vi "Measurement Logic.vi"() -> ()   [LabVIEW 2022 SP3, in "Noise Sweep_Class D Amplifier.lvlib"]
uses:
  Noise Sweep_Class D Amplifier.lvlib
  <vilib>/Analysis/NI_AALBase.lvlib
  <instrlib>/niDCPower/nidcpower.llb/niDCPower Source Mode.ctl
  <instrlib>/niDCPower/nidcpower.llb/niDCPower Output Function.ctl
  Measurement Results.ctl
  <instrlib>/niDCPower/nidcpower.llb/niDCPower Wait For Event - Event.ctl
  <vilib>/Analysis/NI_AALPro.lvlib
  shared/DAQmx/DAQmx utility.lvlib
  shared/digital serial api/Digital Serial.lvclass
  shared/digital serial gen settings/digital audio protocol controls.lvlib
  shared/controls/digital output level units.ctl
  shared/controls/audio controls.lvlib
  service/generation/controls/sine wave properties.ctl
  service/generation/controls/AudioGenTypeDefs.lvlib
  shared/controls/weighting filter.ctl
  shared/controls/highpass filter.ctl
  shared/controls/lowpass filter.ctl
  shared/controls/audio filter settings.ctl
  <vilib>/DAQmx/configure/timing.llb/DAQmx Timing (Sample Clock).vi
  <vilib>/DAQmx/create/channels.llb/DAQmx Create Channel (AI-Voltage-Basic).vi
  <vilib>/Analysis/1siggen.llb/Ramp Pattern by Samples.vi
  <vilib>/Analysis/5stat.llb/RMS (DBL).vi
  <vilib>/Plug-In SDKs/Measurements/Measure Call Context/Measure Call Context.lvclass
  Measurement Configuration.ctl
  shared/DAQmx/input terminal configuration.ctl
panel:
  out "XY Graph":cluster{"X data":dbl[], "Y data":dbl[]}[](graph)
  out "Waveform Graph":waveform(dbl)[](graph)
  out "measure call context out":refnum<class "Measure Call Context.lvclass">
  in  "measure call context in":refnum<class "Measure Call Context.lvclass">
  out "measurement results":T1={"channel names"=[], "power supply voltage (V)"=[], "idle channel noise (Vrms)"=[], "wfm - dt"=1.9531249997269942e-05, "wfm - data"=array[12800 elements]}
  in  "measurement configuration":T2={"digital serial cfg file"="", "digital channel list"="7821\\PCMo 8", "master clock channel list"="7821\\PCMo 0", "acq channel"="PXI1Slot4/ai0", "acq sampling rate"=51200.0, "measurement time (s)"=0.1, "delay before measurement (s)"=0.1, "input range"=5.0, "input terminal cfg"=enum."Default", "weighting filter"=enum."A-weighting", "lowpass filter"=enum."No filter", "highpass filter"=enum."DC", "power supply resource"="PXI1Slot6", "power supply voltage start"=5.0, "power supply voltage stop"=14.0, "sweep number of steps"=10, "power supply current limit"=1.2}
  out "error out":errorcluster
  in  "error in":errorcluster
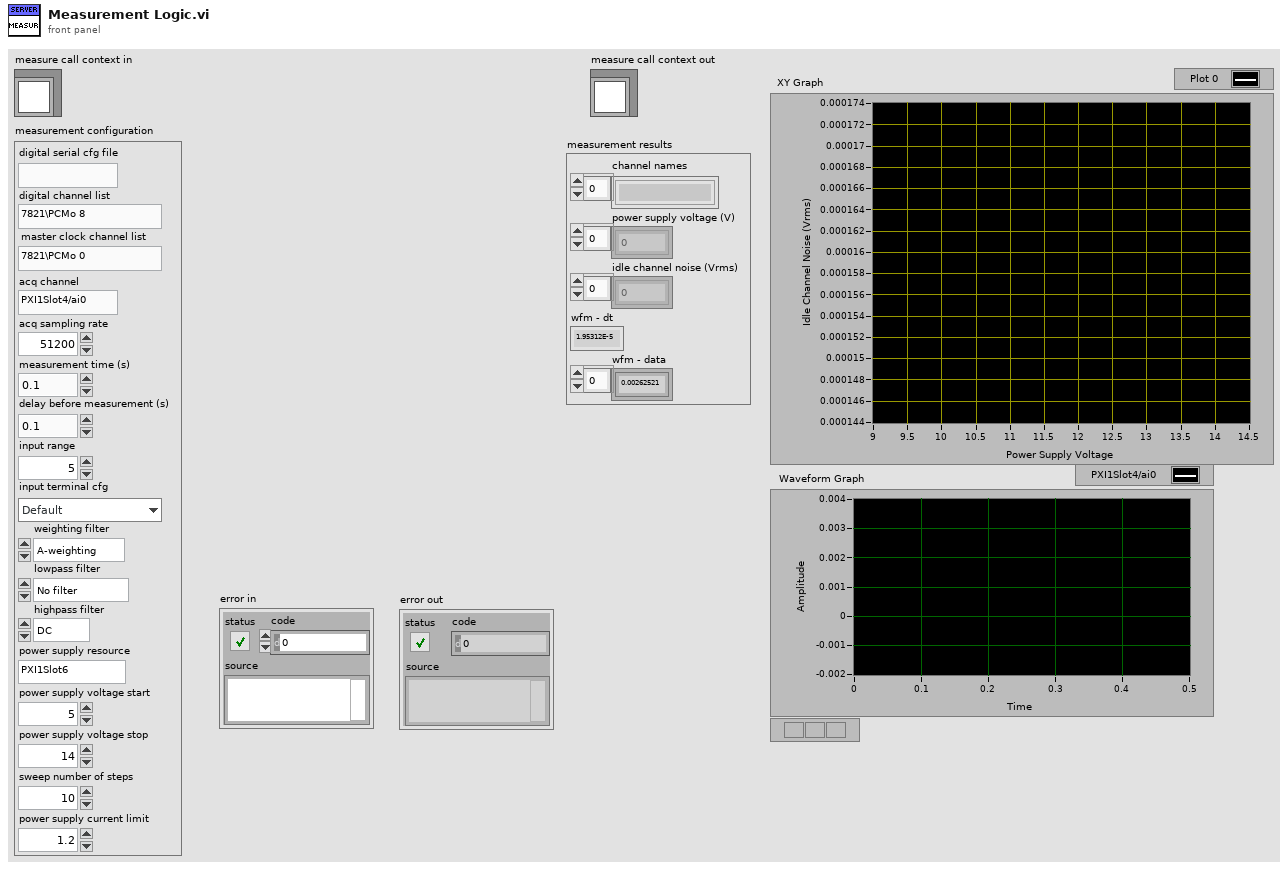
[diagram p1: front panel]
types:
  T1 = typedef "Noise Sweep_Class D Amplifier.lvlib/Measurement Results.ctl" = cluster{"channel names":string[], "power supply voltage (V)":dbl[], "idle channel noise (Vrms)":dbl[], "wfm - dt":dbl, "wfm - data":dbl[]}
  T2 = typedef "Noise Sweep_Class D Amplifier.lvlib/Measurement Configuration.ctl" = cluster{"digital serial cfg file":string, "digital channel list":string, "master clock channel list":string, "acq channel":string, "acq sampling rate":dbl, "measurement time (s)":dbl, "delay before measurement (s)":dbl, "input range":dbl, "input terminal cfg":T3, "weighting filter":T4, "lowpass filter":T5, "highpass filter":T6, "power supply resource":string, "power supply voltage start":dbl, "power supply voltage stop":dbl, "sweep number of steps":u32, "power supply current limit":dbl}
  T3 = typedef "DAQmx utility.lvlib/input terminal configuration.ctl" = enum32{"Default", "NRSE", "RSE", "Differential", "Pseudodifferential"}
  T4 = typedef "weighting filter.ctl" = enum32{"Linear", "A-weighting", "B-weighting", "C-weighting"}
  T5 = typedef "lowpass filter.ctl" = enum32{"No filter", "AES17 20kHz", "AES17 40kHz"}
  T6 = typedef "highpass filter.ctl" = enum32{"DC", "AC"}
  T7 = typedef "audio filter settings.ctl" = cluster{"weighting filter":T4, "highpass filter":T6, "lowpass filter ":T5}
  T8 = typedef "AudioGenTypeDefs.lvlib/sine wave properties.ctl" = cluster{"frequency":dbl, "amplitude":dbl, "phase":dbl}[]
  T9 = typedef "audio controls.lvlib/digital output level units.ctl" = enum32{"% FS", "dBFS", "V"}
  T10 = typedef "niDCPower Output Function.ctl" = i32
  T11 = typedef "niDCPower Source Mode.ctl" = i32
  T12 = typedef "digital serial gen settings.ctl" = cluster{"number of channels":u32, "data justification":T13, "endianness":T14, "channel length":u32, "bit depth":u32, "frame clock rate":dbl, "bit clock edge sync":T15, "master clock rate":dbl, "Logic Level":T16, "frame sync edge for channel 0":T15, "Channel 0 Offset":u32}
  T13 = typedef "PDM Shared.lvlib/PCM Data Justification.ctl" = enum16{"Left Justified", "Right Justified"}
  T14 = typedef "PDM Shared.lvlib/PCM Bit Endianness.ctl" = enum16{"MSB First", "LSB First"}
  T15 = typedef "PDM Shared.lvlib/Digital Edge.ctl" = enum8{"Rising", "Falling"}
  T16 = typedef "PDM Acquisition Class Library.lvlib/DecoderSession.lvclass/Logic Levels.ctl" = enum16{"3.3 V", "1.8 V", "1.2 V"}
  T17 = typedef "AudioGenTypeDefs.lvlib/digital protocol settings.ctl" = cluster{"logic level":T16, "PCM Data Configuration":T18, "bit clock rate":sgl, "master clock rate":sgl, "clock mode":T19, "Frame Sync Clock Control":T20}
  T18 = typedef "PDM Shared.lvlib/PCM Data Format Configuration.ctl" = cluster{"Frame Sync Edge for Channel 0":T15, "Channel Count Per Frame":u8, "Channel Length":u16, "Bit Depth":u8, "Channel 0 Offset":u16, "Endianness":T14, "Data Justification":T13}
  T19 = typedef "PDM Shared.lvlib/clock mode.ctl" = enum16{"divided clock", "DDS"}
  T20 = typedef "PDM Shared.lvlib/PCM Frame Sync Control.ctl" = cluster{"Frame Length":u16, "Frame Sync Pulse Width":u16, "Bit Clock Edge  Sync":T15}
  T21 = typedef "niDCPower Wait For Event - Event.ctl" = i32
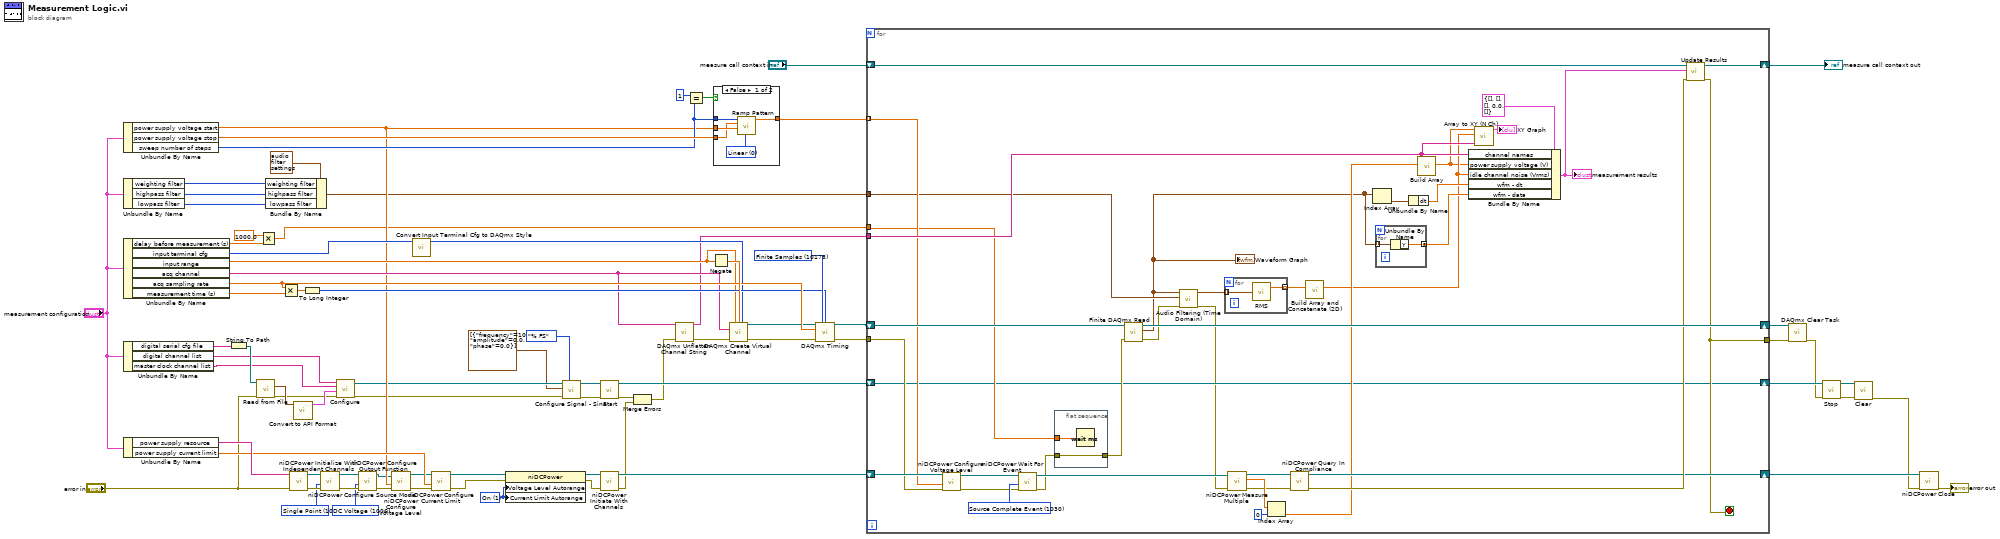
[diagram p0: block diagram]
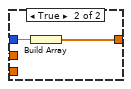
[diagram p2: hidden frame]
diagram:
  w33 = 1 items=["Off", "On"] ("Source:DC Voltage:Current Limit Autorange")
  w34 = T10 1006 items=["DC Voltage"=1006, "DC Current"=1007, "Pulse Voltage"=1049, "Pulse Current"=1050] ("output function")
  w41 = T11 1020 items=["Single Point"=1020, "Sequence"=1021] ("source mode")
  w65 = 10178 items=["Finite Samples"=10178, "Continuous Samples"=10123, "Hardware Timed Single Point"=12522] ("sample mode")
  n1 = Unbundle By Name("measurement configuration") -> ("power supply voltage start"=w49:dbl, "power supply voltage stop"=w68:dbl, "sweep number of steps"=w67:u32)
  n2 = Unbundle By Name("measurement configuration") -> ("weighting filter"=w4:T4, "highpass filter"=w3:T6, "lowpass filter"=w2:T5)
  n3 = Unbundle By Name("measurement configuration") -> ("delay before measurement (s)"=w32:dbl, "input terminal cfg"=w57:T3, "input range"=w59:dbl, "acq channel"=w51:string, "acq sampling rate"=w63:dbl, "measurement time (s)"=w64:dbl)
  n4 = Unbundle By Name("measurement configuration") -> ("digital serial cfg file"=w26:string, "digital channel list"=w19:string, "master clock channel list"=w18:string)
  n5 = Unbundle By Name("measurement configuration") -> ("power supply resource"=w73:string, "power supply current limit"=w72:dbl)
  n6 = String To Path(string=w26) -> (path=w25:path)
  n7 = call "Read from File.vi"("error in (no error)"="error in", "file path"=w25) -> ("error out"=w24:errorcluster, "digital audio protocol settings"=w29:T12)  [unwired: 7 in, 1 out]
  n8 = Multiply(x=1000.0, y=w32) -> (x*y=w30:dbl)
  n9 = Bundle By Name(cluster=T7 {"weighting filter"=enum."C-weighting", "highpass filter"=enum."AC", "lowpass filter "=enum."AES17 20kHz"} ("filter settings"), "weighting filter"=w4, "highpass filter"=w3, "lowpass filter"=w2) -> (w1:T7)
  n10 = Multiply(x=w63, y=w64) -> (x*y=w62:dbl)
  n11 = call <instrlib>:"niDCPower Initialize With Independent Channels.vi"("error in (no error)"="error in", "resource name"=w73) -> ("error out"=w45:errorcluster, "instrument handle out"=w44:refnum<k15>)  [unwired: 8 in]
  n12 = call "Convert to API Format.vi"("digital audio protocol settings"=w29) -> ("digital protocol settings"=w28:T17)  [unwired: 10 in]
  n13 = To Long Integer(number=w62) -> (32bit integer=w61:i32)
  n14 = call <instrlib>:"niDCPower Configure Source Mode.vi"("error in (no error)"=w45, "source mode"=w41, "instrument handle"=w44) -> ("error out"=w43:errorcluster, "instrument handle out"=w42:refnum<k15>)  [unwired: 7 out]
  n15 = call "Configure.vi"("error in (no error)"=w24, "digital protocol settings"=w28, "master clock channel list"=w18, "data channel list"=w19) -> ("error out"=w23:errorcluster, "digital serial task"=w22:refnum<class "Digital Serial.lvclass">)  [unwired: 6 in]
  n16 = call <instrlib>:"niDCPower Configure Output Function.vi"("error in (no error)"=w43, "output function"=w34, "instrument handle"=w42) -> ("error out"=w35:errorcluster, "instrument handle out"=w36:refnum<k15>)  [unwired: 1 in, 6 out]
  n17 = call <instrlib>:"niDCPower Configure Voltage Level.vi"("error in (no error)"=w35, "voltage level"=w49, "instrument handle"=w36) -> ("error out"=w46:errorcluster, "instrument handle out"=w47:refnum<k15>)  [unwired: 1 in, 6 out]
  n18 = call "Convert Input Terminal Cfg to DAQmx Style.vi"("input terminal cfg"=w57) -> ("DAQmx input terminal cfg"=w58:i32)  [unwired: 10 in]
  n19 = call <instrlib>:"niDCPower Configure Current Limit.vi"("error in (no error)"=w46, "current limit"=w72, "instrument handle"=w47) -> ("error out"=w37:errorcluster, "instrument handle out"=w40:refnum<k15>)  [unwired: 2 in, 5 out]
  n20 = property class="niDCPower"(reference=w40, error in=w37, "Voltage Level Autorange"=w33, "Current Limit Autorange"=w33) -> (reference out=w39:refnum<k15>, error out=w38:errorcluster)
  n21 = call "Configure Signal - Sine.vi"("output level units"=digital_output_level_units."% FS", "error in (no error)"=w23, "sine wave properties"=T8 [{"frequency"=1000.0, "amplitude"=0.0, "phase"=0.0}], "Digital Serial in"=w22) -> ("error out"=w20:errorcluster, "Digital Serial out"=w21:refnum<class "Digital Serial.lvclass">)  [unwired: 6 in]
  n22 = call <instrlib>:"niDCPower Initiate With Channels.vi"("error in (no error)"=w38, "instrument handle"=w39) -> ("error out"=w16:errorcluster, "instrument handle out"=w48:refnum<k15>)  [unwired: 8 in]
  n23 = call "Start.vi"("error in (no error)"=w20, "Digital Serial in"=w21) -> ("error out"=w15:errorcluster, "Digital Serial out"=w17:refnum<class "Digital Serial.lvclass">)  [unwired: 8 in]
  n24 = Merge Errors(w15, w16) -> (w14:errorcluster)
  n25 = call <vilib>:"DAQmx Unflatten Channel String.vi"("names in"=w51, "error in"=w14) -> ("names out"=w50:string[], "error out"=w52:errorcluster)  [unwired: 12 in]
  n26 = Equal?(x=u32 1, y=w67) -> (x = y?=w76:bool)
  n27 = Negate(x=w59) -> (-x=w66:dbl)
  n28 = case shown="False" w76 {
    tunnel: w49 -> [w83 w85]
    tunnel: w68 -> [w82 _]
    tunnel: w67 -> [w81 _]
    tunnel: [w80 w84] -> w78
    frame False {
      w79 = u16 0 items=["Linear", "Logarithmic"] ("type")
      n29 = call-poly <vilib>:"Ramp Pattern.vi"("type"=w79, "start"=w83, "end"=w82, "samples"=w81) -> ("Ramp Pattern"=w80:dbl[])  [unwired: 6 in, 1 out]
    }
    frame True {
      n30 = Build Array(w85) -> (w84:dbl[])
    }
  }
  n31 = call-poly <vilib>:"DAQmx Create Virtual Channel.vi"("maximum value"=w59, "minimum value"=w66, "input terminal configuration"=w58, "physical channels"=w51, "error in"=w52) -> ("task out"=w56:refnum<k21>, "error out"=w55:errorcluster)  [unwired: 9 in]
  n32 = call-poly <vilib>:"DAQmx Timing.vi"("task/channels in"=w56, "sample mode"=w65, "samples per channel"=w61, "rate"=w63, "error in"=w55) -> ("task out"=w54:refnum<k21>, "error out"=w53:errorcluster)  [unwired: 9 in]
  n33 = for {
    tunnel: w78 -> [w99] mode=indexing
    shift-right: [w123] -> w77
    shift-left: "measure call context in" -> [w122]
    shift-right: [w112] -> w70
    shift-left: w48 -> [w117]
    shift-right: [w120] -> w69
    shift-left: w54 -> [w119]
    tunnel: w53 -> [w116]
    tunnel: [w111] -> w60
    tunnel: w50 -> [w105]
    tunnel: w30 -> [w92]
    shift-right: [w91] -> w13
    shift-left: w17 -> [w91]
    tunnel: w1 -> [w87]
    stop <- w111 stop-if-true
    w115 = T21 1030 items=["Source Complete Event"=1030, "Measure Complete Event"=1031, "Sequence Iteration Complete Event"=1032, "Sequence Engine Done Event"=1033] ("event")
    n34 = call <instrlib>:"niDCPower Configure Voltage Level.vi"("error in (no error)"=w116, "voltage level"=w99, "instrument handle"=w117) -> ("error out"=w97:errorcluster, "instrument handle out"=w98:refnum<k15>)  [unwired: 1 in, 6 out]
    n35 = call <instrlib>:"niDCPower Wait For Event.vi"("error in (no error)"=w97, "event"=w115, "instrument handle"=w98) -> ("error out"=w101:errorcluster, "instrument handle out"=w114:refnum<k15>)  [unwired: 1 in, 6 out]
    n36 = flat-sequence {
      tunnel: w101 -> [w125]
      tunnel: [w125] -> w100
      tunnel: w92 -> [w124]
      frame #0 {
        n37 = Wait (ms)(milliseconds to wait=w124) -> ()  [unwired: 1 out]
      }
    }
    n38 = call "Finite DAQmx Read.vi"("error in (no error)"=w100, "task/channels in"=w119) -> ("error out"=w89:errorcluster, "data"=w86:waveform(dbl)[], "task out"=w120:refnum<k21>)  [unwired: 7 in]
    "Waveform Graph" <- w86
    n39 = call "Audio Filtering (Time Domain).vi"("waveforms"=w86, "filter settings"=w87, "error in"=w89) -> ("time domain"=w90:waveform(dbl)[], "error out"=w88:errorcluster)  [unwired: 6 in]
    n40 = for {
      tunnel: w90 -> [w129] mode=indexing
      tunnel: [w128] -> w106 mode=indexing
      n41 = call-poly <vilib>:"RMS.vi"("X"=w129) -> ("rms value"=w128:dbl)  [unwired: 1 out]
    }
    n42 = call <instrlib>:"niDCPower Measure Multiple.vi"("error in (no error)"=w88, "instrument handle"=w114) -> ("error out"=w94:errorcluster, "voltage measurements"=w95:dbl[], "instrument handle out"=w93:refnum<k15>)  [unwired: 6 in, 1 out]
    n43 = Index Array(array=w95, index=0) -> (element=w109:dbl)
    n44 = call <instrlib>:"niDCPower Query In Compliance.vi"("error in (no error)"=w94, "instrument handle"=w93) -> ("error out"=w113:errorcluster, "instrument handle out"=w112:refnum<k15>)  [unwired: 1 in, 7 out]
    n45 = call "Build Array and Concatenate (2D).vi"("Array"=w106) -> ("Array Out"=w103:dbl[])  [unwired: 10 in]
    n46 = Index Array(array=w86) -> (element=w110:waveform(dbl))  [unwired: 1 in]
    n47 = for {
      tunnel: w86 -> [w127] mode=indexing
      tunnel: [w126] -> w107 mode=concatenating
      n48 = Unbundle By Name(w127) -> ("Y"=w126:dbl[])
    }
    n49 = Unbundle By Name(w110) -> ("dt"=w108:dbl)
    n50 = call "Build Array.vi"("value"=w109) -> ("Array"=w102:dbl[])  [unwired: 10 in]
    n51 = Bundle By Name(cluster=T1 {"channel names"=[], "power supply voltage (V)"=[], "idle channel noise (Vrms)"=[], "wfm - dt"=0.0, "wfm - data"=[]} ("Measurement Results"), "channel names"=w105, "power supply voltage (V)"=w102, "idle channel noise (Vrms)"=w103, "wfm - dt"=w108, "wfm - data"=w107) -> (w121:T1)
    "measurement results" <- w121
    n52 = call "Array to XY (N Ch).vi"("channel names"=w105, "Y data"=w103, "X data"=w102) -> ("XY plots"=→"XY Graph":cluster{"X data":dbl[], "Y data":dbl[]}[])  [unwired: 8 in]
    n53 = call <vilib>:"Update Results.vi"("error in"=w113, "measurement results"=w121, "measure call context in"=w122) -> ("error out"=w111:errorcluster, "measure call context out"=w123:refnum<class "Measure Call Context.lvclass">)  [unwired: 7 in]
  }
  "measure call context out" <- w77
  n54 = call <vilib>:"DAQmx Clear Task.vi"("task in"=w69, "error in"=w60) -> ("error out"=w12:errorcluster)  [unwired: 13 in]
  n55 = call "Stop.vi"("error in (no error)"=w12, "Digital Serial in"=w13) -> ("error out"=w11:errorcluster, "Digital Serial out"=w10:refnum<class "Digital Serial.lvclass">)  [unwired: 8 in]
  n56 = call "Clear.vi"("error in (no error)"=w11, "Digital Serial in"=w10) -> ("error out"=w9:errorcluster)  [unwired: 9 in]
  n57 = call <instrlib>:"niDCPower Close.vi"("error in (no error)"=w9, "instrument handle"=w70) -> ("error out"=→"error out":errorcluster)  [unwired: 9 out]
